vi "set Limit Line Setting.vi"(8 "error in (no error)":errorcluster, 9 "Turn On?":bool, 10 "Limit Line Setting":T1={"Limit Line Index"=1, "Frequency Table"=[], "Amplitude Table"=[], "Name"=""} {"Limit Line Index" min=1 max=8}, 11 "FSV-40N in":refnum<class "FSV-40N.lvclass">) -> (0 "error out":errorcluster, 3 "FSV-40N out":refnum<class "FSV-40N.lvclass">)   [LabVIEW 2023, in "Spectrum Analyzer.lvlib" / "FSV-40N.lvclass"]
uses:
  FSV-40N.lvclass
  TYPE DEFINITION/TYPE Limit Line Setting Table.ctl
  FSV-40N.lvclass/FSV-40N.ctl
  Spectrum Analyzer.lvlib
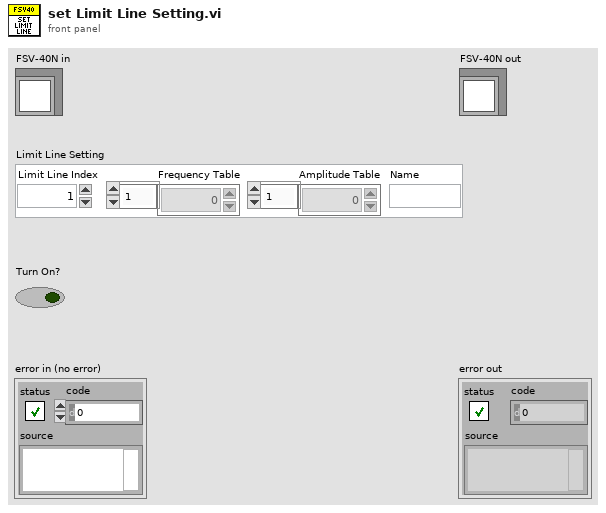
[diagram p1: front panel]
types:
  T1 = typedef "Spectrum Analyzer.lvlib/TYPE Limit Line Setting Table.ctl" = cluster{"Limit Line Index":i32, "Frequency Table":dbl[], "Amplitude Table":dbl[], "Name":string}
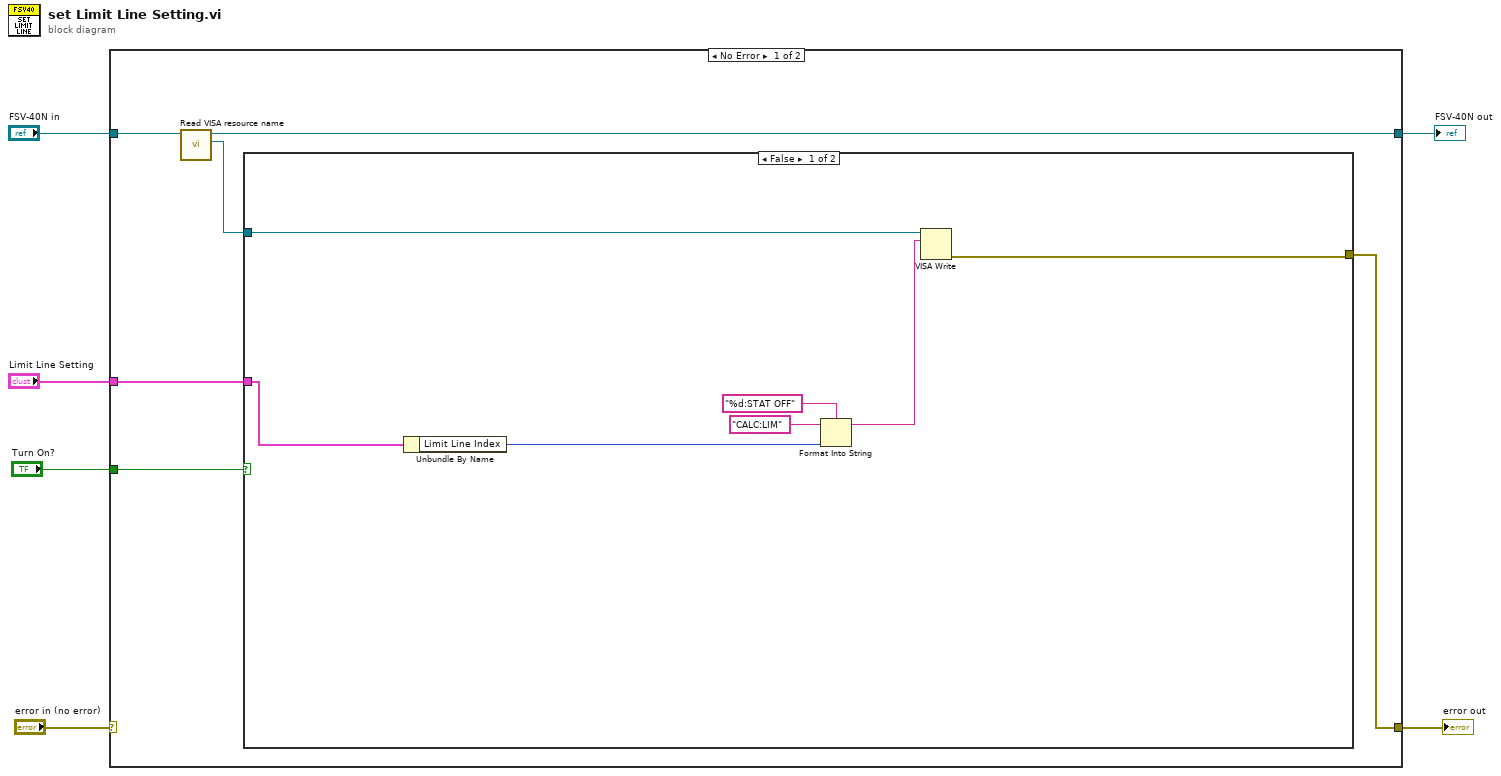
[diagram p0: block diagram]
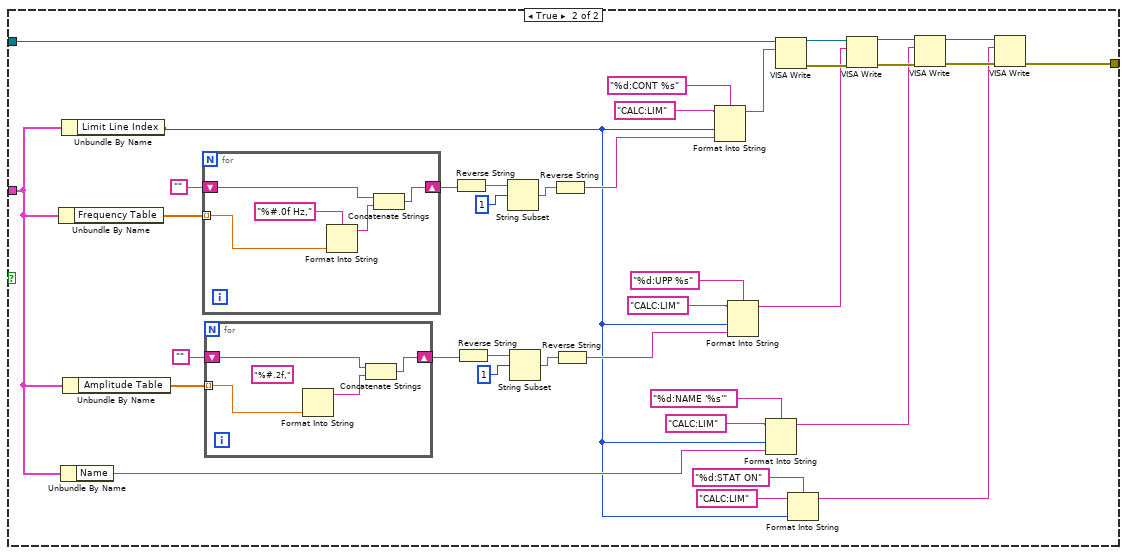
[diagram p2: hidden frame]
diagram:
  n1 = case shown="No Error" "error in (no error)" {
    selector: "error in (no error)" -> [_ w66]
    tunnel: "FSV-40N in" -> [w12 w67]
    tunnel: [w11 w67] -> w4
    tunnel: [w7 w66] -> w3
    tunnel: "Limit Line Setting" -> [w8 _]
    tunnel: "Turn On?" -> [w10 _]
    frame No Error {
      n2 = call "Read VISA resource name.vi"("FSV-40N in"=w12) -> ("VISA resource name"=w9:refnum<visa-resource-name>, "FSV-40N out"=w11:refnum<class "FSV-40N.lvclass">)  [unwired: 8 in, 1 out]
      n3 = case shown="False" w10 {
        tunnel: w9 -> [w15 w44]
        tunnel: w8 -> [w17 w41]
        tunnel: [w13 w20] -> w7
        frame False {
          n4 = Unbundle By Name(w17) -> ("Limit Line Index"=w16:i32)
          n5 = Format Into String(format string="%d:STAT OFF", initial string="CALC:LIM", w16) -> (resulting string=w14:string)  [unwired: 1 in, 1 out]
          n6 = VISA Write(VISA resource name=w15, write buffer=w14) -> (error out=w13:errorcluster)  [unwired: 1 in, 2 out]
        }
        frame True {
          n7 = Unbundle By Name(w41) -> ("Frequency Table"=w56:dbl[])
          n8 = Unbundle By Name(w41) -> ("Name"=w38:string)
          n9 = Unbundle By Name(w41) -> ("Limit Line Index"=w26:i32)
          n10 = Unbundle By Name(w41) -> ("Amplitude Table"=w45:dbl[])
          n11 = for {
            tunnel: w56 -> [w61] mode=indexing
            shift-right: [w64] -> w54
            shift-left: "" -> [w65]
            n12 = Format Into String(format string="%#.0f Hz,", w61) -> (resulting string=w62:string)  [unwired: 2 in, 1 out]
            n13 = Concatenate Strings(w65, w62) -> (w64:string)
          }
          n14 = for {
            tunnel: w45 -> [w58] mode=indexing
            shift-right: [w59] -> w47
            shift-left: "" -> [w60]
            (unwired) "%#.2f," ("format string")
            n15 = Format Into String(w58) -> (resulting string=w57:string)  [unwired: 3 in, 1 out]
            n16 = Concatenate Strings(w60, w57) -> (w59:string)
          }
          n17 = Reverse String(1:w54) -> (0:w53:string)
          n18 = Reverse String(1:w47) -> (0:w48:string)
          n19 = String Subset(string=w53, offset (0)=1) -> (substring=w51:string)  [unwired: 1 in]
          n20 = String Subset(string=w48, offset (0)=1) -> (substring=w50:string)  [unwired: 1 in]
          n21 = Reverse String(1:w51) -> (0:w28:string)
          n22 = Reverse String(1:w50) -> (0:w32:string)
          n23 = Format Into String(format string="%d:CONT %s", initial string="CALC:LIM", w26, w28) -> (resulting string=w27:string)  [unwired: 1 in, 1 out]
          n24 = Format Into String(format string="%d:UPP %s", initial string="CALC:LIM", w26, w32) -> (resulting string=w31:string)  [unwired: 1 in, 1 out]
          n25 = Format Into String(format string="%d:NAME '%s'", initial string="CALC:LIM", w26, w38) -> (resulting string=w35:string)  [unwired: 1 in, 1 out]
          n26 = VISA Write(VISA resource name=w44, write buffer=w27) -> (VISA resource name out=w43:refnum<visa-resource-name>, error out=w42:errorcluster)  [unwired: 1 in, 1 out]
          n27 = Format Into String(format string="%d:STAT ON", initial string="CALC:LIM", w26) -> (resulting string=w21:string)  [unwired: 1 in, 1 out]
          n28 = VISA Write(VISA resource name=w43, write buffer=w31, error in (no error)=w42) -> (VISA resource name out=w37:refnum<visa-resource-name>, error out=w36:errorcluster)  [unwired: 1 out]
          n29 = VISA Write(VISA resource name=w37, write buffer=w35, error in (no error)=w36) -> (VISA resource name out=w23:refnum<visa-resource-name>, error out=w22:errorcluster)  [unwired: 1 out]
          n30 = VISA Write(VISA resource name=w23, write buffer=w21, error in (no error)=w22) -> (error out=w20:errorcluster)  [unwired: 2 out]
        }
      }
    }
    frame Error {
    }
  }
  "error out" <- w3
  "FSV-40N out" <- w4
